vi "VIH HelpGen - Image - Add Transparency to Icon Picture.vi"(9 "Source Color (white)":u32=16777215 format="%.0x", 11 "2D Picture":picture) -> (3 "2D Picture out":picture)   [LabVIEW 2014]
doc: "::: VI Helpeks :::\nCopyright (c) 2000-2026 Konstantin Shifershteyn. All rights reserved."
panel:
  # "VI Helpeks\nCopyright (c) 2012-2026 Konstantin Shifershteyn"
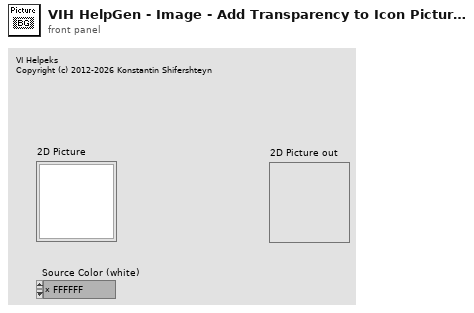
[diagram p1: front panel]
types:
  T1 = typedef "imagedata.ctl" = cluster{"image type":i32, "image depth":i32, "image":u8[], "mask":u8[], "colors":u32[], "Rectangle":cluster{"left":i16, "top":i16, "right":i16, "bottom":i16}}
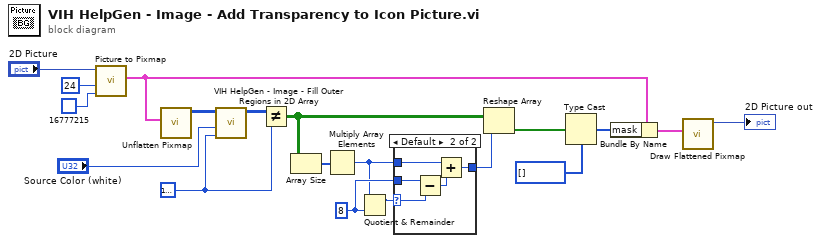
[diagram p0: block diagram]
diagram:
  w7 = 8 ("y")
  w1 = u32 16777216
  n1 = call <vilib>:"Picture to Pixmap.vi"("Background Color"=u32 16777215, "depth"=24, "picture"="2D Picture") -> ("image data"=w16:T1)  [unwired: 7 in, 1 out]
  n2 = call <vilib>:"Unflatten Pixmap.vi"("image data"=w16) -> ("24-bit pixmap"=w4:u32[][])  [unwired: 4 in, 6 out]
  n3 = call "VIH HelpGen - Image - Fill Outer Regions in 2D Array.vi"("New Color (transparent)"=w1, "Source Color (white)"="Source Color (white)", "Image Data in"=w4) -> ("Image Data out"=w3:u32[][])  [unwired: 8 in]
  n4 = Not Equal?(x=w3, y=w1) -> (x != y?=w12:bool[][])
  n5 = Array Size(array=w12) -> (size(s)=w13:i32[])
  n6 = Multiply Array Elements(1:w13) -> (0:w6:i32)
  n7 = Quotient & Remainder(x=w6, y=w7) -> (x-y*floor(x/y)=w8:i32)  [unwired: 1 out]
  n8 = case shown="Default" w8 {
    selector: w8 -> [_ w21]
    tunnel: w6 -> [w20 w25]
    tunnel: w7 -> [_ w24]
    tunnel: [w20 w22] -> w5
    frame 0 {
    }
    frame Default {
      n9 = Subtract(x=w24, y=w21) -> (x-y=w23:i32)
      n10 = Add(x=w25, y=w23) -> (x+y=w22:i32)
    }
  }
  n11 = Reshape Array(w12, w5) -> (w10:bool[])
  n12 = Type Cast(type=u8[] [], x=w10) -> (*(type *) &x=w9:u8[])
  n13 = Bundle By Name(cluster=w16, "mask"=w9) -> (w14:T1)
  n14 = call <vilib>:"Draw Flattened Pixmap.vi"("image data"=w14) -> ("new picture"=→"2D Picture out":picture)  [unwired: 8 in]
